vi "路灯仿真_B站参考版V2.vi"() -> ()   [LabVIEW 2014]
panel:
  out "计时器 2":dbl
  out "绿 2":bool
  out "黄 2":bool
  out "红 2":bool
  in  "布尔":bool
  out "计时器":dbl
  out "绿":bool
  out "黄":bool
  out "红":bool
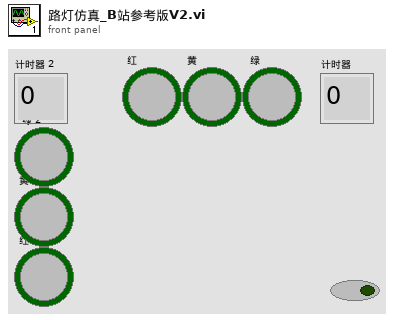
[diagram p1: front panel]
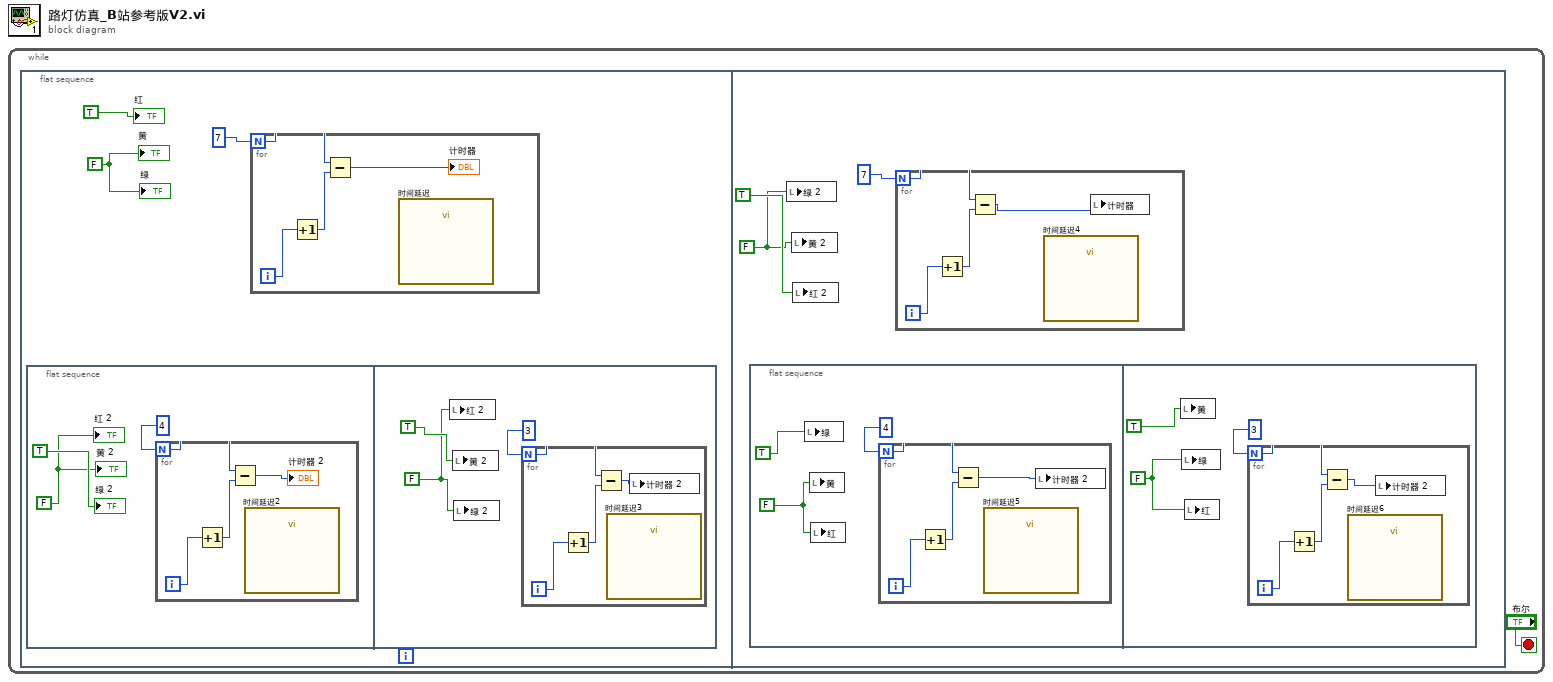
[diagram p0: block diagram]
diagram:
  n1 = while {
    stop <- "布尔" stop-if-true
    n2 = flat-sequence {
      frame #0 {
        w3 = FALSE
        n3 = flat-sequence {
          frame #0 {
            w6 = FALSE
            n4 = for {
              N: 4 -> [w9]
              i -> [w11]
              n5 = Increment(x=w11) -> (x+1=w10:i32)
              n6 = Subtract(x=w9, y=w10) -> (x-y=→"计时器 2":i32)
              n7 = call "时间延迟2"() -> ()  [unwired: 11 in, 1 out]
            }
            "黄 2" <- w6
            "绿 2" <- TRUE
            "红 2" <- w6
          }
          frame #1 {
            w13 = FALSE
            n8 = local write "红 2"(w13) -> ()
            n9 = local write "黄 2"(TRUE) -> ()
            n10 = local write "绿 2"(w13) -> ()
            n11 = for {
              N: 3 -> [w16]
              i -> [w18]
              n12 = Increment(x=w18) -> (x+1=w17:i32)
              n13 = Subtract(x=w16, y=w17) -> (x-y=w15:i32)
              n14 = call "时间延迟3"() -> ()  [unwired: 11 in, 1 out]
              n15 = local write "计时器 2"(w15) -> ()
            }
          }
        }
        n16 = for {
          N: 7 -> [w20]
          i -> [w22]
          n17 = Increment(x=w22) -> (x+1=w21:i32)
          n18 = Subtract(x=w20, y=w21) -> (x-y=→"计时器":i32)
          n19 = call "时间延迟"() -> ()  [unwired: 11 in, 1 out]
        }
        "红" <- TRUE
        "黄" <- w3
        "绿" <- w3
      }
      frame #1 {
        w23 = FALSE
        n20 = flat-sequence {
          frame #0 {
            w26 = FALSE
            n21 = local write "绿"(TRUE) -> ()
            n22 = local write "黄"(w26) -> ()
            n23 = local write "红"(w26) -> ()
            n24 = for {
              N: 4 -> [w30]
              i -> [w32]
              n25 = Increment(x=w32) -> (x+1=w31:i32)
              n26 = Subtract(x=w30, y=w31) -> (x-y=w29:i32)
              n27 = call "时间延迟5"() -> ()  [unwired: 11 in, 1 out]
              n28 = local write "计时器 2"(w29) -> ()
            }
          }
          frame #1 {
            w34 = FALSE
            n29 = local write "黄"(TRUE) -> ()
            n30 = local write "绿"(w34) -> ()
            n31 = local write "红"(w34) -> ()
            n32 = for {
              N: 3 -> [w37]
              i -> [w39]
              n33 = Increment(x=w39) -> (x+1=w38:i32)
              n34 = Subtract(x=w37, y=w38) -> (x-y=w36:i32)
              n35 = call "时间延迟6"() -> ()  [unwired: 11 in, 1 out]
              n36 = local write "计时器 2"(w36) -> ()
            }
          }
        }
        n37 = local write "绿 2"(w23) -> ()
        n38 = local write "黄 2"(w23) -> ()
        n39 = local write "红 2"(TRUE) -> ()
        n40 = for {
          N: 7 -> [w41]
          i -> [w43]
          n41 = Increment(x=w43) -> (x+1=w42:i32)
          n42 = Subtract(x=w41, y=w42) -> (x-y=w40:i32)
          n43 = call "时间延迟4"() -> ()  [unwired: 11 in, 1 out]
          n44 = local write "计时器"(w40) -> ()
        }
      }
    }
  }
